vi "libssh2_session_supported_algs.vi"(8 "error in (no error)":errorcluster, 10 "method_type":T1, 11 "session":T2) -> (0 "error out":errorcluster, 2 "algs":string[](array[string]))   [LabVIEW 2017, in "libssh2.lvlib"]
doc: "Get the supported algorithms for a method type.\n\nFor a list of supported compression algorithms, <B>libssh2_session_flag</B> must be called with LIBSSH2_FLAG_COMPRESS=1. Otherwise, \"none\" will be returned.\n\nIf successful, returns an array with supported algorithms as defined in RFC 4253."
uses:
  libssh2.lvlib
  Session Refnum.ctl
  libssh2_method_type.ctl
  Not A Session.vi
  <vilib>/Utility/error.llb/Error Cluster From Error Code.vi
  Global Settings.vi
  Read Session Refnum.vi
  <vilib>/Utility/semaphor.llb/Acquire Semaphore.vi
  <vilib>/Utility/semaphor.llb/Release Semaphore.vi
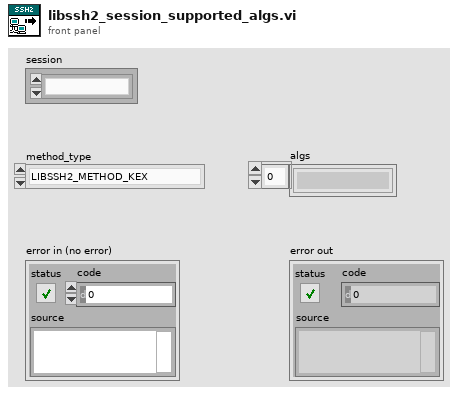
[diagram p1: front panel]
types:
  T1 = typedef "libssh2.lvlib/libssh2_method_type.ctl" = enum16{"LIBSSH2_METHOD_KEX", "LIBSSH2_METHOD_HOSTKEY", "LIBSSH2_METHOD_CRYPT_CS", "LIBSSH2_METHOD_CRYPT_SC", "LIBSSH2_METHOD_MAC_CS", "LIBSSH2_METHOD_MAC_SC", "LIBSSH2_METHOD_COMP_CS", "LIBSSH2_METHOD_COMP_SC", "LIBSSH2_METHOD_LANG_CS", "LIBSSH2_METHOD_LANG_SC", "LIBSSH2_METHOD_SIGN_ALGO"}
  T2 = typedef "libssh2.lvlib/Session Refnum.ctl" = refnum<k1>
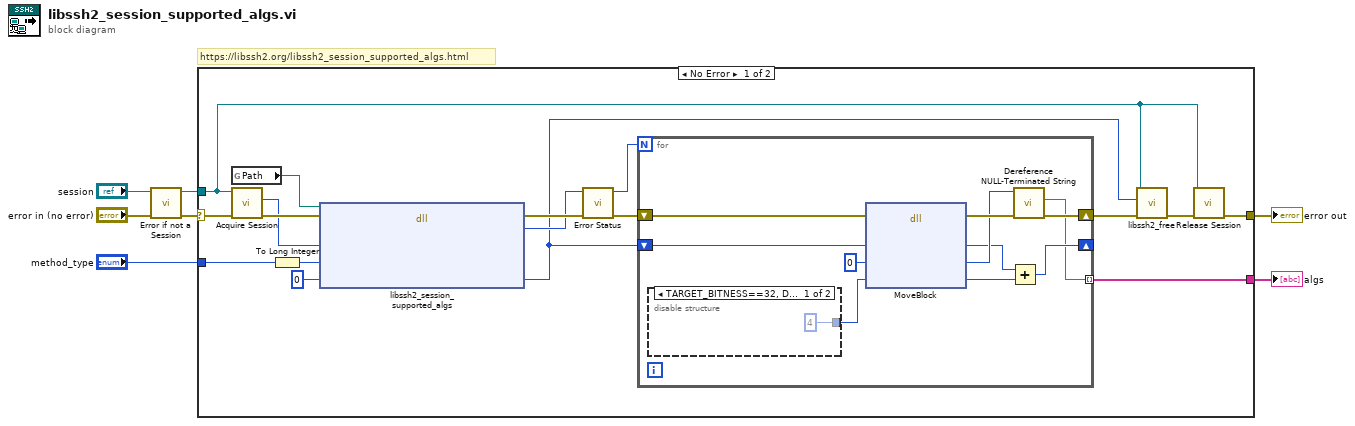
[diagram p0: block diagram]
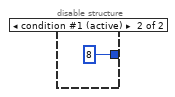
[diagram p2: hidden frame]
diagram:
  # "https://libssh2.org/libssh2_session_supported_algs.html"
  n1 = call "Error if not a Session.vi"("error in (no error)"="error in (no error)", "session"="session") -> ("error out"=w5:errorcluster, "session out"=w3:T2)  [unwired: 8 in]
  n2 = case shown="No Error" w5 {
    selector: w5 -> [w23 w38]
    tunnel: [w9 w38] -> w7
    tunnel: w3 -> [w8 _]
    tunnel: "method_type" -> [w19 _]
    tunnel: [w11 _] -> w1
    frame No Error {
      n3 = global read "Global Settings.vi" "Path"() -> (w20:path)
      n4 = call "Acquire Session.vi"("error in (no error)"=w23, "session"=w8) -> ("error out"=w22:errorcluster, "LIBSSH2_SESSION*"=w21:u64)  [unwired: 7 in, 1 out]
      n5 = To Long Integer(number=w19) -> (32bit integer=w18:i32)
      n6 = dll-call lib="?" fn="libssh2_session_supported_algs"(path in=w20, error in=w22, "session"=w21, "method_type"=w18, "algs"=u64 0) -> (error out=w24:errorcluster, "return value"=w17:i32, "algs"=w10:u64)  [unwired: 3 in, 1 out]
      n7 = call "Error Status.vi"("error in (no error)"=w24, "return value"=w17) -> ("error out"=w15:errorcluster, "return value out"=w12:i32)  [unwired: 8 in]
      n8 = for {
        N: w12 -> [_]
        shift-right: [w32] -> w14
        shift-left: w15 -> [w35]
        shift-right: [w30] -> _
        shift-left: w10 -> [w31]
        tunnel: [w29] -> w11 mode=indexing
        n9 = disable-structure shown="TARGET_BITNESS==32, Default" {
          disable-tunnel: [i64 4 ("size") i64 8 ("size")] -> w27
          frame condition #0 {
          }
          frame condition #1 (active) {
          }
        }
        n10 = dll-call lib="LabVIEW" fn="MoveBlock"(error in=w35, "ps"=w31, "pd"=u64 0, "size"=w27) -> (error out=w34:errorcluster, "ps"=w26:u64, "pd"=w33:u64, "size"=w25:i64)  [unwired: 3 in, 1 out]
        n11 = Add(x=w26, y=w25) -> (x+y=w30:u64)
        n12 = call "Dereference NULL-Terminated String.vi"("error in (no error)"=w34, "char*"=w33) -> ("error out"=w32:errorcluster, "string"=w29:string)  [unwired: 8 in]
      }
      n13 = call "libssh2_free.vi"("error in (no error)"=w14, "ptr"=w10, "session"=w8) -> ("error out"=w13:errorcluster)  [unwired: 8 in]
      n14 = call "Release Session.vi"("error in (no error)"=w13, "session"=w8) -> ("error out"=w9:errorcluster)  [unwired: 9 in]
    }
    frame Error {
    }
  }
  "error out" <- w7
  "algs" <- w1
